vi "Test Status Rate.vi"() -> ()   [LabVIEW 2021]
uses:
  CAN RW CANsub.lvclass
  <vilib>/CIF Foundation/CIF CAN RW Core/typedef/CAN Mode.ctl
  <vilib>/CIF Foundation/CIF CAN RW Core/CAN_RW_CORE.lvclass
  <vilib>/CIF Foundation/CIF CAN RW Core/typedef/FD Config.ctl
  <vilib>/CIF Foundation/CIF CAN RW Core/typedef/CAN Port Configuration.ctl
panel:
  out "error out":errorcluster
  out "iterations":i32
  in  "run time (s)":u32=10
  in  "interface":string="192.168.0.49/2"
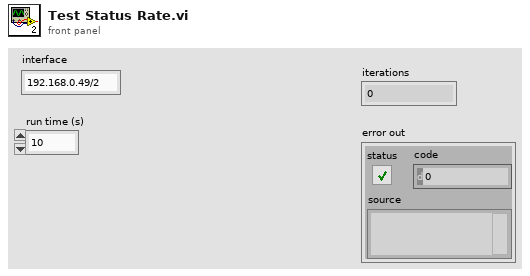
[diagram p1: front panel]
types:
  T1 = typedef "CAN_RW_CORE.lvclass/CAN Port Configuration.ctl" = cluster{"Mode":T2, "Baud Rate":u64, "Temination On":bool, "Subordinate":bool, "Echo TX":bool, "FD Config":T3}
  T2 = typedef "CAN_RW_CORE.lvclass/CAN Mode.ctl" = enum16{"CAN 2.0", "CAN FD"}
  T3 = typedef "CAN_RW_CORE.lvclass/FD Config.ctl" = cluster{"FD Baud Rate":u64, "ISO Mode":bool, "BRS Enabled":bool}
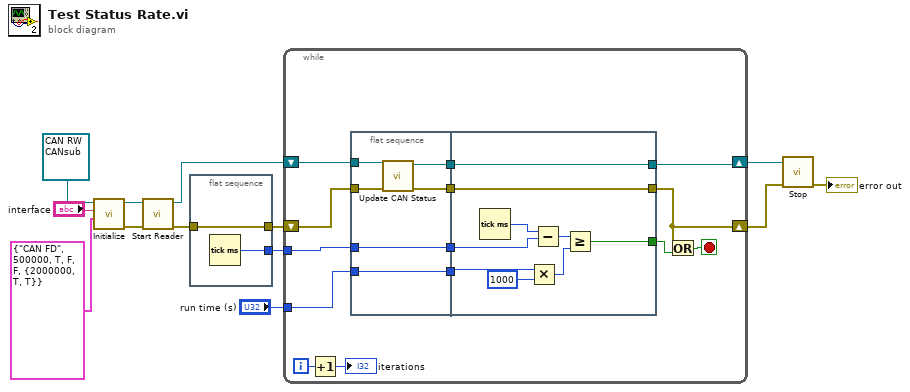
[diagram p0: block diagram]
diagram:
  n1 = call "Initialize.vi"("Port Configuration"=T1 {"Mode"=enum."CAN FD", "Baud Rate"=500000, "Temination On"=TRUE, "Subordinate"=FALSE, "Echo TX"=FALSE, "FD Config"={"FD Baud Rate"=2000000, "ISO Mode"=TRUE, "BRS Enabled"=TRUE}}, "Interface"="interface", "CANsub_CAN_RW in"=refnum<class "CAN RW CANsub.lvclass"> refnum) -> ("error out"=w2:errorcluster, "CANsub_CAN_RW out"=w11:refnum<class "CAN RW CANsub.lvclass">)  [unwired: 7 in]
  n2 = call-dynamic "Start Reader.vi"("error in (no error)"=w2, "CAN RW CANsub in"=w11) -> ("error out"=w13:errorcluster, "CAN RW CANsub out"=w9:refnum<class "CAN RW CANsub.lvclass">)  [unwired: 8 in]
  n3 = flat-sequence {
    tunnel: w13 -> [w14]
    tunnel: [w15] -> w12
    tunnel: [w14] -> w8
    frame #0 {
      n4 = Tick Count (ms)() -> (millisecond timer value=w15:u32)
    }
  }
  n5 = while {
    tunnel: w12 -> [w25]
    shift-right: [w19] -> w6
    shift-left: w9 -> [w28]
    shift-right: [w17] -> w5
    shift-left: w8 -> [w27]
    tunnel: "run time (s)" -> [w23]
    i -> [w29]
    stop <- w20 stop-if-true
    n6 = Increment(x=w29) -> (x+1=→"iterations":i32)
    n7 = flat-sequence {
      tunnel: w28 -> [w35]
      tunnel: w27 -> [w34]
      tunnel: [w33] -> w26
      tunnel: w25 -> [w33]
      tunnel: [w32] -> w24
      tunnel: w23 -> [w32]
      tunnel: [w31] -> w22
      tunnel: [w30] -> w18
      tunnel: w26 -> [w43]
      tunnel: w24 -> [w42]
      tunnel: [w38] -> w17
      tunnel: w22 -> [w38]
      tunnel: [w37] -> w21
      tunnel: [w36] -> w19
      tunnel: w18 -> [w36]
      frame #0 {
        n8 = call "Update CAN Status.vi"("error in (no error)"=w34, "CAN RW CANsub in"=w35) -> ("error out"=w31:errorcluster, "CAN RW CANsub out"=w30:refnum<class "CAN RW CANsub.lvclass">)  [unwired: 8 in]
      }
      frame #1 {
        n9 = Tick Count (ms)() -> (millisecond timer value=w44:u32)
        n10 = Multiply(x=w42, y=u32 1000) -> (x*y=w39:u32)
        n11 = Subtract(x=w44, y=w43) -> (x-y=w40:u32)
        n12 = Greater Or Equal?(x=w40, y=w39) -> (x >= y?=w37:bool)
      }
    }
    n13 = Or(x=w17, y=w21) -> (x .or. y?=w20:bool)
  }
  n14 = call-dynamic "Stop.vi"("error in (no error)"=w5, "CAN RW CANsub in"=w6) -> ("error out"=→"error out":errorcluster)  [unwired: 8 in, 1 out]
